vi "Load Transition Config.vi"(8 "error in (no error)":refnum<class "MultiErrors.lvclass">, 10 "Config Element":refnum<class "Config Element.lvclass">, 11 "State Transition Config in":refnum<class "State Transition Config.lvclass">) -> (0 "error out":refnum<class "MultiErrors.lvclass">, 3 "State Transition Config out":refnum<class "State Transition Config.lvclass">)   [LabVIEW 2020, in "VolatusSeqConfig.lvlib" / "State Transition Config.lvclass"]
uses:
  State Transition Config.lvclass
  VolatusErrorUtilities/MultiErrors/MultiErrors.lvclass
  lv-cdm/CDM-Config/Config Element/Config Element.lvclass
  State Transition Config.lvclass/State Transition Config.ctl
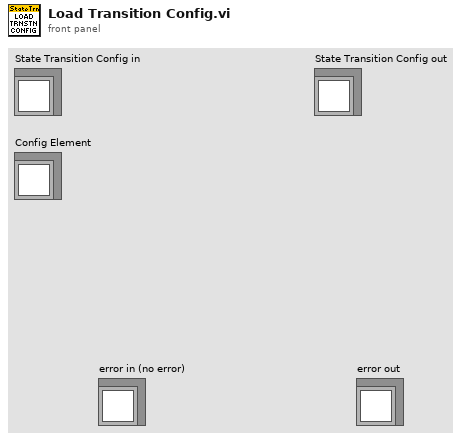
[diagram p1: front panel]
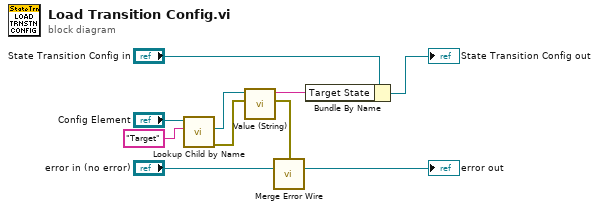
[diagram p0: block diagram]
diagram:
  n1 = call "Lookup Child by Name.vi"("Name"="Target", "Config Element in"="Config Element") -> ("error out"=w3:errorcluster, "Child"=w6:refnum<class "Config Element.lvclass">)  [unwired: 6 in, 2 out]
  n2 = call "Value (String).vi"("error in (no error)"=w3, "Config Element in"=w6) -> ("error out"=w1:errorcluster, "String Value"=w4:string)  [unwired: 8 in]
  n3 = call "Merge Error Wire.vi"("error in (no error)"=w1, "MultiErrors in"="error in (no error)") -> ("MultiErrors out"=→"error out":refnum<class "MultiErrors.lvclass">)  [unwired: 13 in]
  n4 = Bundle By Name(cluster="State Transition Config in", "Target State"=w4) -> (→"State Transition Config out":refnum<class "State Transition Config.lvclass">)
